vi "Draw Curves.vi"(11 "Data Viewer in":refnum<class "Data Viewer.lvclass">) -> (1 "Scale Visible":bool[](array[boolean]), 3 "Data Viewer Out":refnum<class "Data Viewer.lvclass">)   [LabVIEW 2020, in "Data Viewer.lvlib" / "Data Viewer.lvclass"]
uses:
  Data Viewer.lvclass
  Legend.ctl
  Data Viewer.lvclass/Data Viewer.ctl
  2d3f1c39-fb65-4b1e-85c3-c2b4405b819a.vi
  <vilib>/Comparison/Equal/Equal Functor/Equal Functor.lvclass
  Data Viewer.lvlib
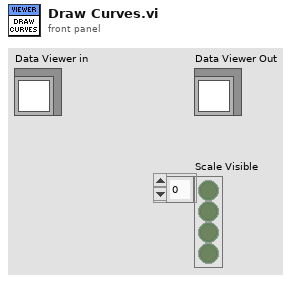
[diagram p1: front panel]
types:
  T1 = typedef "Data Viewer.lvlib/Data Viewer.lvclass/Legend.ctl" = cluster{"颜色":u32, "曲线名称":string}[]
  T2 = cluster{"Plot Index":i32, "Scale Index":i32, "Color":u32, "Peak Line?":bool}
  T3 = typedef "Data Viewer.lvlib/Data Viewer.lvclass/Plot Property--cluster.ctl" = cluster{"Name":string, "Visible":bool, "Color":u32, "Scale Index":i32, "Show Peak Line":bool}
  T4 = typedef "Data Viewer.lvlib/Data Serie--cluster.ctl" = cluster{"Name":string, "Unit":string, "Sample Rate[Hz]":dbl, "Delta t[S]":dbl, "t0":timestamp, "Length":i32, "Time":timestamp[], "Value":dbl[]}
  T5 = cluster{"Plot Index":i32, "Scale Index":i32, "Color":u32, "Peak Line?":bool}[]
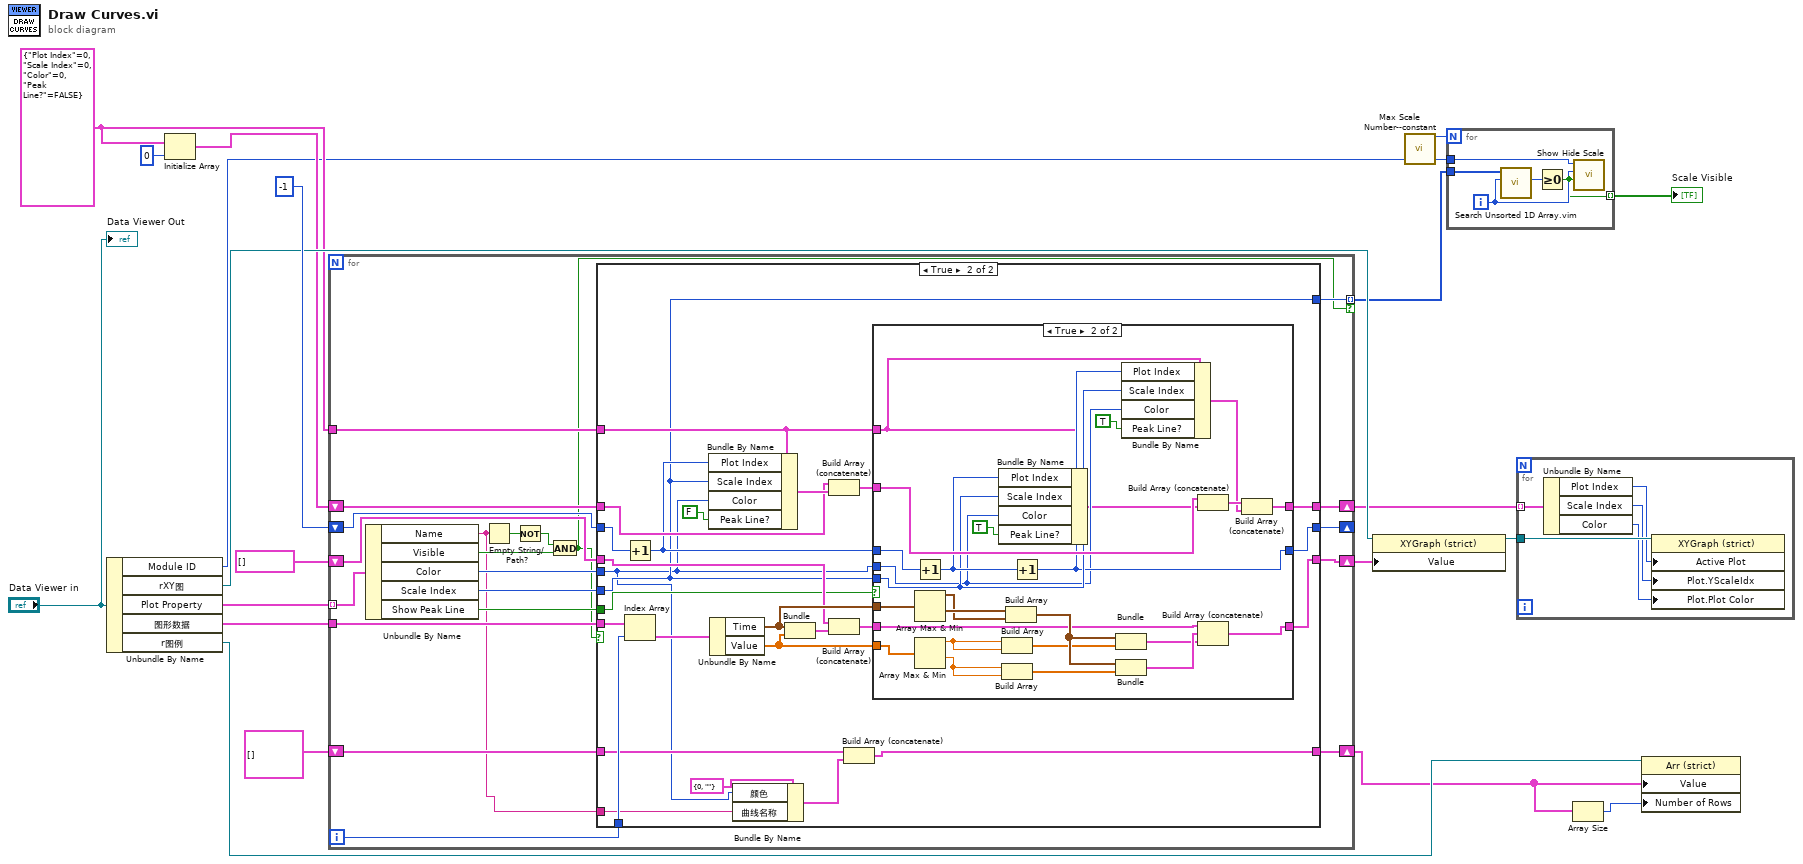
[diagram p0: block diagram]
diagram:
  w12 = T2 {"Plot Index"=0, "Scale Index"=0, "Color"=0, "Peak Line?"=FALSE}
  n1 = Unbundle By Name("Data Viewer in") -> ("Module ID"=w6:i32, "rXY图"=w15:refnum<vi>, "Plot Property"=w19:T3[], "图形数据"=w18:T4[], "r图例"=w4:refnum<vi>)
  n2 = Initialize Array(w12, 0 ("dimension size")) -> (w10:T5)
  n3 = for {
    tunnel: w19 -> [w41] mode=indexing
    tunnel: w18 -> [w37]
    shift-right: [w30] -> w14
    shift-left: cluster{"Time":timestamp[], "Value":dbl[]}[] [] -> [w36]
    shift-right: [w27] -> w9
    shift-left: w10 -> [w34]
    shift-right: [w31] -> _
    shift-left: -1 -> [w35]
    tunnel: w12 -> [w29]
    tunnel: [w26] -> w7 mode=indexing if=w25
    shift-right: [w21] -> w3
    shift-left: T1 [] ("图例") -> [w23]
    i -> [w24]
    n4 = Unbundle By Name(w41) -> ("Name"=w22:string, "Visible"=w38:bool, "Color"=w28:u32, "Scale Index"=w33:i32, "Show Peak Line"=w32:bool)
    n5 = Empty String/Path?(string/path=w22) -> (empty?=w40:bool)
    n6 = Not(x=w40) -> (.not. x?=w39:bool)
    n7 = And(x=w39, y=w38) -> (x .and. y?=w25:bool)
    n8 = case shown="True" w25 {
      tunnel: w37 -> [_ w71]
      tunnel: w36 -> [w45 w67]
      tunnel: w35 -> [w43 w65]
      tunnel: w34 -> [w44 w63]
      tunnel: w33 -> [_ w53]
      tunnel: w32 -> [_ w62]
      tunnel: [w43 w60] -> w31
      tunnel: [w44 w59] -> w27
      tunnel: [w45 w57] -> w30
      tunnel: w29 -> [_ w56]
      tunnel: w28 -> [_ w49]
      tunnel: [_ w53] -> w26
      tunnel: w24 -> [_ w52]
      tunnel: w23 -> [w42 w51]
      tunnel: w22 -> [_ w48]
      tunnel: [w42 w46] -> w21
      frame False {
      }
      frame True {
        n9 = Increment(x=w65) -> (x+1=w54:i32)
        n10 = Index Array(array=w71, index=w52) -> (element=w70:T4)
        n11 = Bundle By Name(cluster=w56, "Plot Index"=w54, "Scale Index"=w53, "Color"=w49, "Peak Line?"=FALSE) -> (w64:T2)
        n12 = Unbundle By Name(w70) -> ("Time"=w69:timestamp[], "Value"=w68:dbl[])
        n13 = Bundle By Name(cluster=cluster{"颜色":u32, "曲线名称":string} {"颜色"=0, "曲线名称"=""} ("簇 2"), "颜色"=w49, "曲线名称"=w48) -> (w47:cluster{"颜色":u32, "曲线名称":string})
        n14 = Bundle("Time"=w69, "Value"=w68) -> (w66:cluster{"Time":timestamp[], "Value":dbl[]})  [unwired: 1 in]
        n15 = Build Array (concatenate)(w63, w64) -> (w61:T5)
        n16 = Build Array (concatenate)(w67, w66) -> (w58:cluster{"Time":timestamp[], "Value":dbl[]}[])
        n17 = Build Array (concatenate)(w51, w47) -> (w46:T1)
        n18 = case shown="True" w62 {
          tunnel: w69 -> [_ w100]
          tunnel: w68 -> [_ w99]
          tunnel: w61 -> [w73 w91]
          tunnel: w54 -> [w72 w90]
          tunnel: w53 -> [_ w87]
          tunnel: [w72 w86] -> w60
          tunnel: [w73 w85] -> w59
          tunnel: w58 -> [w74 w84]
          tunnel: [w74 w81] -> w57
          tunnel: w56 -> [_ w80]
          tunnel: w49 -> [_ w79]
          frame False {
          }
          frame True {
            n19 = Increment(x=w90) -> (x+1=w88:i32)
            n20 = Array Max & Min(array=w100) -> (max value=w97:timestamp, min value=w98:timestamp)  [unwired: 2 out]
            n21 = Array Max & Min(array=w99) -> (max value=w94:dbl, min value=w96:dbl)  [unwired: 2 out]
            n22 = Bundle By Name(cluster=w80, "Plot Index"=w88, "Scale Index"=w87, "Color"=w79, "Peak Line?"=TRUE) -> (w77:T2)
            n23 = Build Array(w94, w94) -> (w92:dbl[])
            n24 = Build Array(w96, w96) -> (w95:dbl[])
            n25 = Build Array(w98, w97) -> (w93:timestamp[])
            n26 = Increment(x=w88) -> (x+1=w86:i32)
            n27 = Bundle(w93, w92) -> (w82:cluster{timestamp[], dbl[]})  [unwired: 1 in]
            n28 = Bundle(w93, w95) -> (w83:cluster{timestamp[], dbl[]})  [unwired: 1 in]
            n29 = Bundle By Name(cluster=w80, "Plot Index"=w86, "Scale Index"=w87, "Color"=w79, "Peak Line?"=TRUE) -> (w78:T2)
            n30 = Build Array (concatenate)(w91, w77) -> (w89:T5)
            n31 = Build Array (concatenate)(w84, w83, w82) -> (w81:cluster{"Time":timestamp[], "Value":dbl[]}[])
            n32 = Build Array (concatenate)(w89, w78) -> (w85:T5)
          }
        }
      }
    }
  }
  n33 = property class="XYGraph (strict)"(reference=w15, "Value"=w14) -> (reference out=w13:refnum<vi>)  [unwired: 1 in, 1 out]
  n34 = call "Max Scale Number--constant.vi"() -> ("Max Scale Number"=w8:i32)  [unwired: 11 in]
  n35 = for {
    N: w8 -> [_]
    tunnel: w7 -> [w105]
    tunnel: w6 -> [w103]
    tunnel: [w101] -> w1 mode=indexing
    i -> [w102]
    n36 = call "Search Unsorted 1D Array.vim"("element"=w102, "unsorted 1D array"=w105) -> ("index of element"=w104:i32)  [unwired: 9 in]
    n37 = Greater Or Equal To 0?(x=w104) -> (x >= 0?=w101:bool)
    n38 = call "Show Hide Scale.vi"("Visible"=w101, "Scale Index"=w102, "Module ID"=w103) -> ()  [unwired: 8 in, 1 out]
  }
  "Scale Visible" <- w1
  n39 = for {
    tunnel: w13 -> [w110]
    tunnel: w9 -> [w109] mode=indexing
    n40 = Unbundle By Name(w109) -> ("Plot Index"=w108:i32, "Scale Index"=w107:i32, "Color"=w106:u32)
    n41 = property class="XYGraph (strict)"(reference=w110, "Active Plot"=w108, "Plot.YScaleIdx"=w107, "Plot.Plot Color"=w106) -> ()  [unwired: 1 in, 2 out]
  }
  n42 = Array Size(array=w3) -> (size(s)=w2:i32)
  n43 = property class="Arr (strict)"(reference=w4, "Value"=w3, "Number of Rows"=w2) -> ()  [unwired: 1 in, 2 out]
  "Data Viewer Out" <- "Data Viewer in"
